vi "VIH Utility - STR - String from 1D Str Array.vi"(6 "delimiter ('\\n')":string="\n", 7 "Array in":string[](array[string])) -> (3 "String out":string)   [LabVIEW 2014]
doc: "::: VI Helpeks :::\nCopyright (c) 2000-2026 Konstantin Shifershteyn. All rights reserved."
panel:
  # "VI Helpeks\nCopyright (c) 2012-2026 Konstantin Shifershteyn"
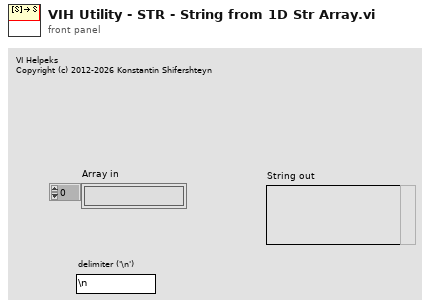
[diagram p1: front panel]
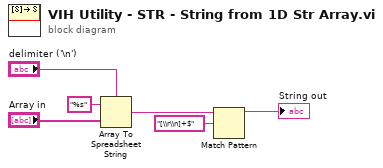
[diagram p0: block diagram]
diagram:
  n1 = Array To Spreadsheet String(delimiter (Tab)="delimiter ('\\n')", array="Array in", 3:"%s" ("format string")) -> (spreadsheet string=w2:string)
  n2 = Match Pattern(string=w2, regular expression="[\\r\\n]+$") -> (before substring=→"String out":string)  [unwired: 4 out]
